vi "REFRIGERANT PRESS TEMP.vi"() -> (2 "Refrigrant Press Tempratures":T1, 3 "Array":dbl[](array[numeric]))   [LabVIEW 2025]
uses:
  <vilib>/Modbus/master/Modbus Master.lvclass
  <vilib>/Modbus/master/Create Master Instance (TCP).vi
panel:
  out "error out":errorcluster
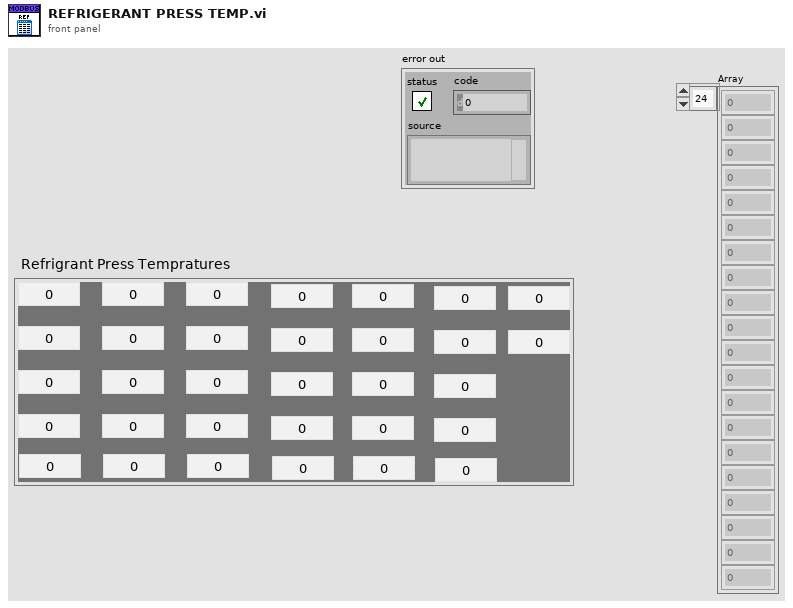
[diagram p1: front panel]
types:
  T1 = cluster{"OFF Coil 1":dbl, "OFF Coil 2":dbl, "OFF Coil 3":dbl, "OFF Coil 4":dbl, "OFF Coil 5":dbl, "OFF Coil 6":dbl, "OFF Coil 7":dbl, "OFF Coil 8":dbl, "OFF Coil 9":dbl, "OFF Coil 10":dbl, "OFF Coil 11":dbl, "OFF Coil 12":dbl, "OFF Coil 13":dbl, "OFF Coil 14":dbl, "OFF Coil 15":dbl, "OFF Coil 16":dbl, "OFF Coil 17":dbl, "OFF Coil 18":dbl, "OFF Coil 19":dbl, "OFF Coil 20":dbl, "OFF Coil 21":dbl, "OFF Coil 22":dbl, "OFF Coil 23":dbl, "OFF Coil 24":dbl, "OFF Coil 25":dbl, "OFF Coil 26":dbl, "OFF Coil 27":dbl, "OFF Coil 28":dbl, "OFF Coil 29":dbl, "OFF Coil 30":dbl, "OFF Coil 31":dbl, "OFF Coil 32":dbl}
  T2 = cluster{"[0]":dbl, "[1]":dbl, "[2]":dbl, "[3]":dbl, "[4]":dbl, "[5]":dbl, "[6]":dbl, "[7]":dbl, "[8]":dbl, "[9]":dbl, "[10]":dbl, "[11]":dbl, "[12]":dbl, "[13]":dbl, "[14]":dbl, "[15]":dbl, "[16]":dbl, "[17]":dbl, "[18]":dbl, "[19]":dbl, "[20]":dbl, "[21]":dbl, "[22]":dbl, "[23]":dbl, "[24]":dbl, "[25]":dbl, "[26]":dbl, "[27]":dbl, "[28]":dbl, "[29]":dbl, "[30]":dbl, "[31]":dbl}
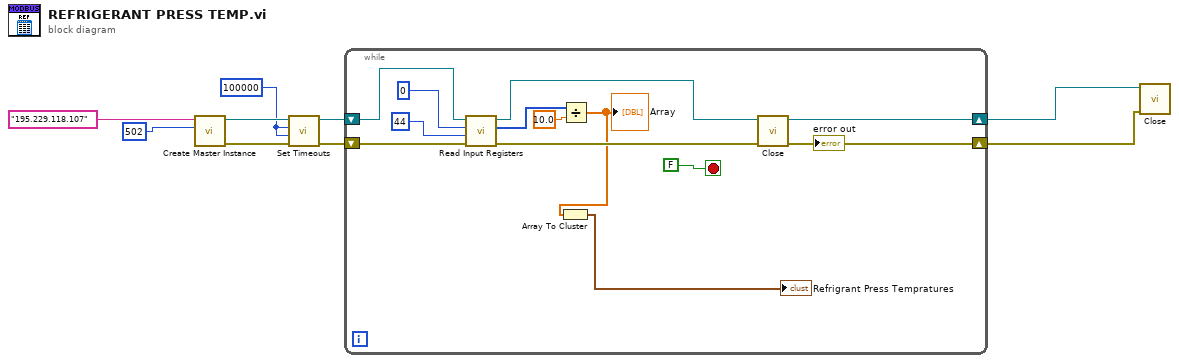
[diagram p0: block diagram]
diagram:
  w3 = 100000 ("read operation timeout (ms)")
  n1 = call-poly <vilib>:"Create Master Instance.vi"("port (502)"=u16 502, "address"="195.229.118.107") -> ("error out"=w4:errorcluster, "TCP master instance"=w5:refnum<class "Modbus Master.lvclass">)  [unwired: 8 in]
  n2 = call <vilib>:"Set Timeouts.vi"("error in (no error)"=w4, "write operation timeout (ms)"=w3, "read operation timeout (ms)"=w3, "Modbus master in"=w5) -> ("error out"=w9:errorcluster, "Modbus master out"=w8:refnum<class "Modbus Master.lvclass">)  [unwired: 6 in]
  n3 = while {
    shift-right: [w21] -> w1
    shift-left: w9 -> [w19]
    shift-right: [w20] -> w2
    shift-left: w8 -> [w18]
    stop <- FALSE stop-if-true
    n4 = call-dynamic "Read Input Registers.vi"("error in (no error)"=w19, "number of input registers"=u16 44, "starting address"=u16 0, "Modbus master in"=w18) -> ("error out"=w21:errorcluster, "register values"=w16:u16[], "Modbus master out"=w20:refnum<class "Modbus Master.lvclass">)  [unwired: 5 in]
    n5 = Divide(x=w16, y=10.0) -> (x/y=w12:dbl[])
    "Array" <- w12
    n6 = Array To Cluster(array=w12) -> (cluster=→"Refrigrant Press Tempratures":T2)
  }
  n7 = call-dynamic "Close.vi"("error in (no error)"=w1, "Modbus master in"=w2) -> ("error out"=→"error out":errorcluster)  [unwired: 9 in]
  n8 = call-dynamic "Close.vi"("error in (no error)"=w1, "Modbus master in"=w2) -> ()  [unwired: 9 in, 1 out]
